vi "cycle_current_output.vi"(0 "Config Parameters":dbl[][](array[numeric]), 5 "Laser Active Ref":refnum<vi>, 7 "Stop Ref":refnum<vi>, 9 "Current Ref":refnum<vi>, 11 "error in":errorcluster) -> (15 "error out":errorcluster)   [LabVIEW 2025, in "tSNIP.lvlib"]
uses:
  tSNIP.lvlib
panel:
  in  "Inc":bool
  out "elapsed time":dbl format="%<%H:%M:%S%1u>t"
  out "Current":cluster{"Value":dbl, "Units":dbl}={"Value"=0.0, "Units"=0.001} {"Units" items=["mA"=0.001, "A"=1.0]; "Value" min=0.0 step=50.0}
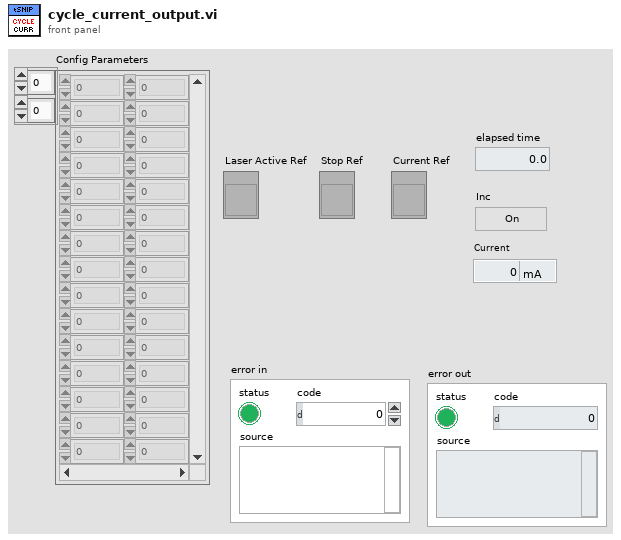
[diagram p1: front panel]
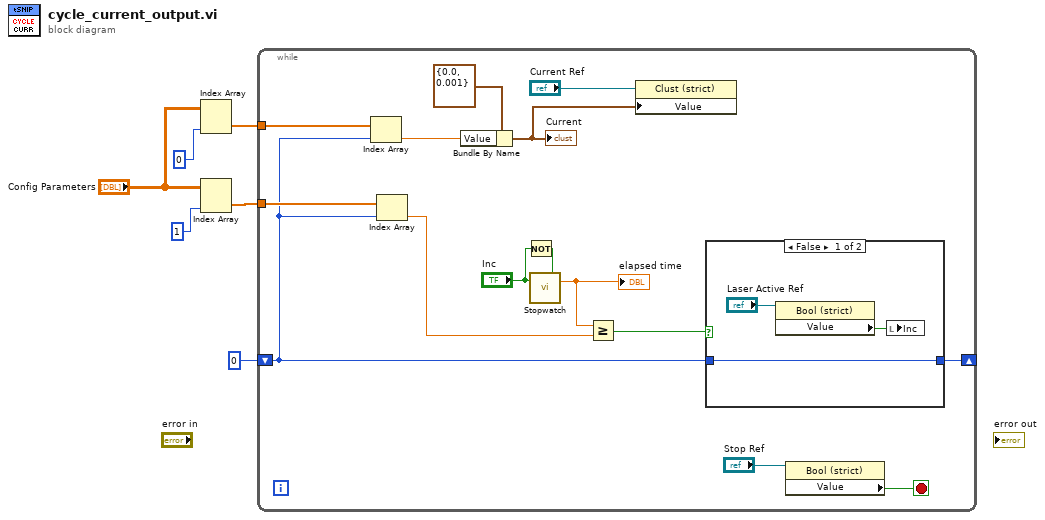
[diagram p0: block diagram]
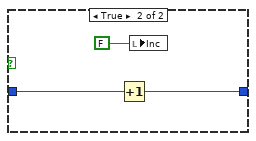
[diagram p2: hidden frame]
diagram:
  n1 = Index Array(array="Config Parameters", index (col)=0) -> (element=w3:dbl[])  [unwired: 1 in]
  n2 = Index Array(array="Config Parameters", index (col)=1) -> (element=w2:dbl[])  [unwired: 1 in]
  n3 = while {
    tunnel: w3 -> [w20]
    tunnel: w2 -> [w19]
    shift-right: [w14] -> _
    shift-left: 0 ("row") -> [w13]
    stop <- w9 stop-if-true
    n4 = Index Array(array=w20, index=w13) -> (element=w18:dbl)
    n5 = Index Array(array=w19, index=w13) -> (element=w15:dbl)
    n6 = Bundle By Name(cluster=cluster{"Value":dbl, "Units":dbl} {"Value"=0.0, "Units"=0.001} ("Current"), "Value"=w18) -> (w7:cluster{"Value":dbl, "Units":dbl})
    "Current" <- w7
    n7 = Not(x="Inc") -> (.not. x?=w21:bool)
    n8 = call "Stopwatch.vi"("Start"="Inc", "Reset"=w21) -> ("time"=w16:dbl)  [unwired: 17 in]
    "elapsed time" <- w16
    n9 = Greater Or Equal?(x=w16, y=w15) -> (x >= y?=w12:bool)
    n10 = property class="Clust (strict)"(reference="Current Ref", "Value"=w7) -> ()  [unwired: 1 in, 2 out]
    n11 = case shown="False" w12 {
      tunnel: w13 -> [w24 w27]
      tunnel: [w24 w26] -> w14
      frame False {
        n12 = property class="Bool (strict)"(reference="Laser Active Ref") -> ("Value"=w22:bool)  [unwired: 1 in, 2 out]
        n13 = local write "Inc"(w22) -> ()
      }
      frame True {
        n14 = Increment(x=w27) -> (x+1=w26:i32)
        n15 = local write "Inc"(FALSE ("Start")) -> ()
      }
    }
    n16 = property class="Bool (strict)"(reference="Stop Ref") -> ("Value"=w9:bool)  [unwired: 1 in, 2 out]
  }
